vi "Add Test Event To Tree.vi"(8 "error in (no error)":errorcluster, 9 "Assert Event Data":T1={"name"="", "passed"=FALSE, "call-chain"=[], "test-error"={"status"=FALSE, "code"=0, "source"=""}, "timestamp"=timestamp(0 s since 1904-01-01), "assert-id"="", "test-id"="", "time"=-1.0, "message"="", "properties"=variant, "measurements"=variant, "user-defined"=variant}, 10 "Parent Key":string, 11 "tree refnum":refnum<vi>) -> (0 "error out":errorcluster, 3 "dup tree refnum":refnum<vi>)   [LabVIEW 2020, in "Caraya.lvlib" / "Basic Test Manager.lvclass"]
uses:
  Basic Test Manager.lvclass
  Test Result/Assert Event Data (Extended).ctl
  Test Result/Test Result.lvclass
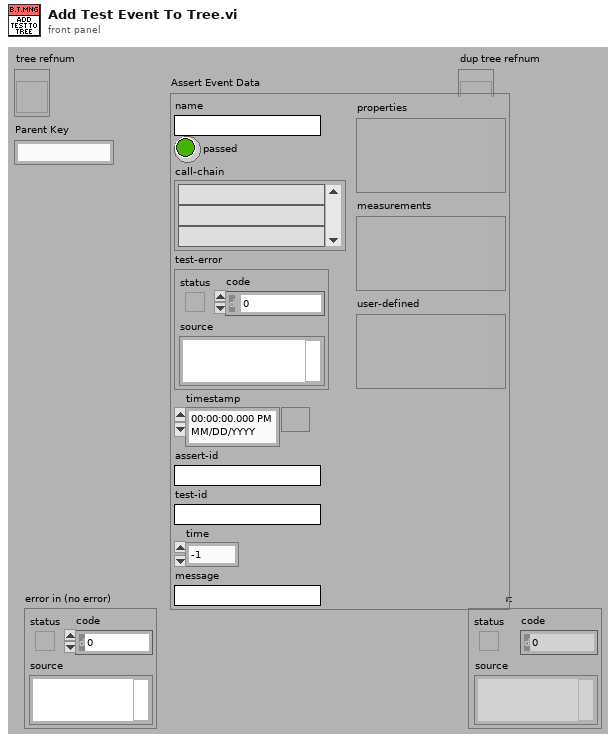
[diagram p1: front panel]
types:
  T1 = typedef "Caraya.lvlib/Test Result.lvclass/Assert Event Data (Extended).ctl" = cluster{"name":string, "passed":bool, "call-chain":string[], "test-error":errorcluster, "timestamp":timestamp, "assert-id":string, "test-id":string, "time":dbl, "message":string, "properties":variant, "measurements":variant, "user-defined":variant}
  T2 = typedef "Caraya.lvlib/Basic Test Manager.lvclass/Test State.ctl" = enum16{"Empty", "Unknown", "Fail", "Pass", "Skip", "Error"}
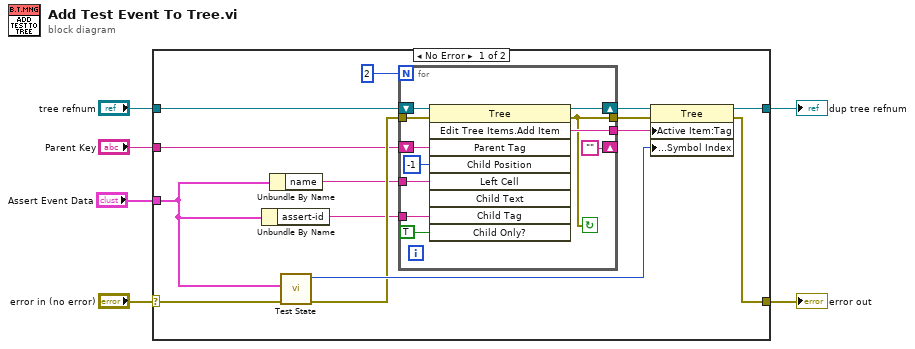
[diagram p0: block diagram]
diagram:
  n1 = case shown="No Error" "error in (no error)" {
    selector: "error in (no error)" -> [w12 w33]
    tunnel: [w14 w33] -> w5
    tunnel: [w18 w32] -> w3
    tunnel: "tree refnum" -> [w20 w32]
    tunnel: "Parent Key" -> [w10 _]
    tunnel: "Assert Event Data" -> [w8 _]
    frame No Error {
      n2 = Unbundle By Name(w8) -> ("assert-id"=w7:string)
      n3 = Unbundle By Name(w8) -> ("name"=w9:string)
      n4 = call "Test State.vi"("error in (no error)"=w12, "Assert Event Data"=w8) -> ("error out"=w11:errorcluster, "Test State"=w16:T2)  [unwired: 8 in]
      n5 = for {
        N: 2 -> [_]
        tunnel: w9 -> [w27]
        tunnel: [w26] -> w17
        shift-right: [w28] -> w19
        shift-left: w20 -> [w31]
        tunnel: w11 -> [w25]
        tunnel: [w24] -> w15
        shift-right: [""] -> _
        shift-left: w10 -> [w30]
        tunnel: w7 -> [w21]
        stop <- w24 continue-if-true
        n6 = invoke on="Invoke Node" class="Tree" method="Edit Tree Items.Add Item"(reference=w31, error in=w25, "Parent Tag"=w30, "Child Position"=-1, "Left Cell"=w27, "Child Tag"=w21, "Child Only?"=TRUE) -> (reference out=w28:refnum<vi>, error out=w24:errorcluster, "Edit Tree Items:Add Item"=w26:string)  [unwired: 2 in, 6 out]
      }
      n7 = property class="Tree"(reference=w19, error in=w15, "Active Item:Tag"=w17, "Active Item:Symbol Index"=w16) -> (reference out=w18:refnum<vi>, error out=w14:errorcluster)
    }
    frame Error {
    }
  }
  "error out" <- w5
  "dup tree refnum" <- w3
